vi "Load Plugins.vi"(8 "error in (no error)":errorcluster, 11 "ChannelManagerUI in":refnum<class "ChannelManagerUI.lvclass">) -> (0 "error out":errorcluster, 3 "ChannelManagerUI out":refnum<class "ChannelManagerUI.lvclass">)   [LabVIEW 2021, in "Channel.lvlib" / "ChannelManagerUI.lvlib" / "ChannelManagerUI.lvclass"]
uses:
  ChannelManagerUI.lvclass
  <vilib>/Utility/file.llb/Read Delimited Spreadsheet (string).vi
  ChannelManagerUI.lvclass/ChannelManagerUI.ctl
  Channel.lvlib
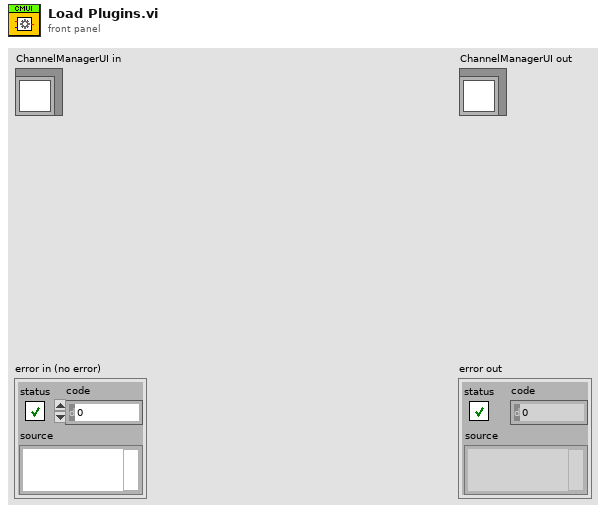
[diagram p1: front panel]
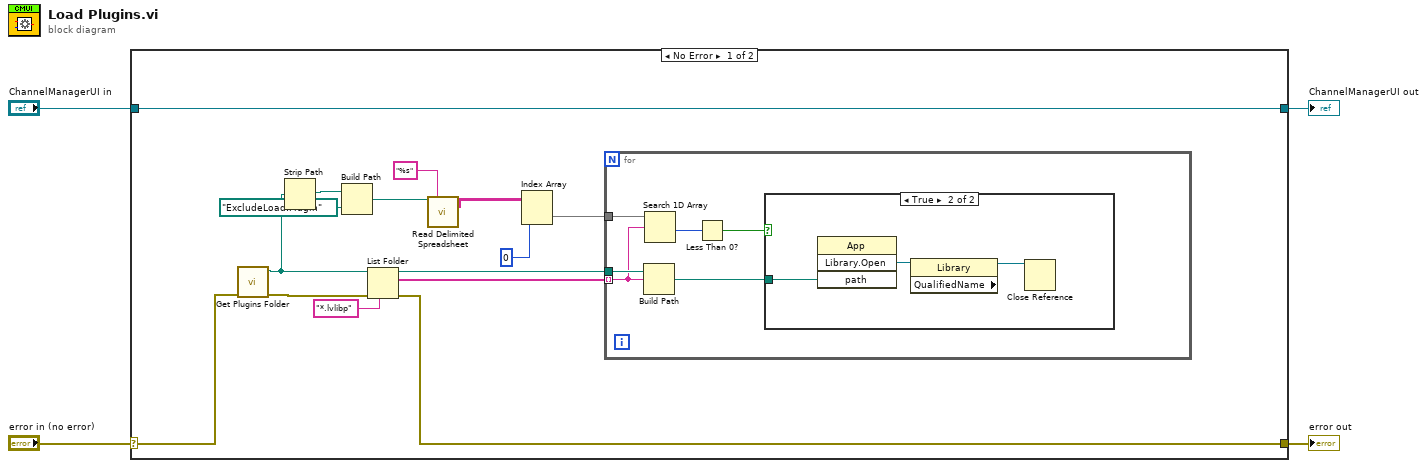
[diagram p0: block diagram]
diagram:
  n1 = case shown="No Error" "error in (no error)" {
    selector: "error in (no error)" -> [w18 w30]
    tunnel: [w16 w30] -> w3
    tunnel: [w19 w29] -> w1
    tunnel: "ChannelManagerUI in" -> [w19 w29]
    frame No Error {
      n2 = call "Get Plugins Folder.vi"("error in (no error)"=w18) -> ("error out"=w17:errorcluster, "Plugins Folder"=w12:path)  [unwired: 9 in]
      n3 = Strip Path(path=w12) -> (stripped path=w11:path)  [unwired: 1 out]
      n4 = Build Path(base path=w11, name or relative path=path "ExcludeLoad.Plugin") -> (appended path=w9:path)
      n5 = List Folder(path=w12, pattern="*.lvlibp", error in=w17) -> (path out=w14:path, filenames=w13:string[], error out=w16:errorcluster)  [unwired: 1 in, 1 out]
      n6 = call-poly <vilib>:"Read Delimited Spreadsheet.vi"("file path (dialog if empty)"=w9, "format (%s)"="%s") -> ("all rows"=w7:string[][])  [unwired: 8 in, 5 out]
      n7 = Index Array(array=w7, index (col)=0 ("disabled index (col)")) -> (element=w5:string[])  [unwired: 1 in]
      n8 = for {
        tunnel: w14 -> [w25]
        tunnel: w13 -> [w22] mode=indexing
        tunnel: w5 -> [w23]
        n9 = Build Path(base path=w25, name or relative path=w22) -> (appended path=w24:path)
        n10 = Search 1D Array(1D array=w23, element=w22) -> (index of element=w21:i32)  [unwired: 1 in]
        n11 = Less Than 0?(x=w21) -> (x < 0?=w20:bool)
        n12 = case shown="True" w20 {
          tunnel: w24 -> [_ w28]
          frame False {
          }
          frame True {
            n13 = invoke class="App" method="Library.Open"("path"=w28) -> ("Open Library"=w27:refnum<vi>)  [unwired: 3 in, 3 out]
            n14 = property class="Library" props=["QualifiedName"](reference=w27) -> (reference out=w26:refnum<vi>)  [unwired: 1 in, 2 out]
            n15 = Close Reference(reference=w26) -> ()  [unwired: 1 in, 1 out]
          }
        }
      }
    }
    frame Error {
    }
  }
  "error out" <- w3
  "ChannelManagerUI out" <- w1
